vi "UMLEditor Main.vi"(1 "StartProject":string, 3 "StartTarget":string) -> ()   [LabVIEW 2020] (continued)
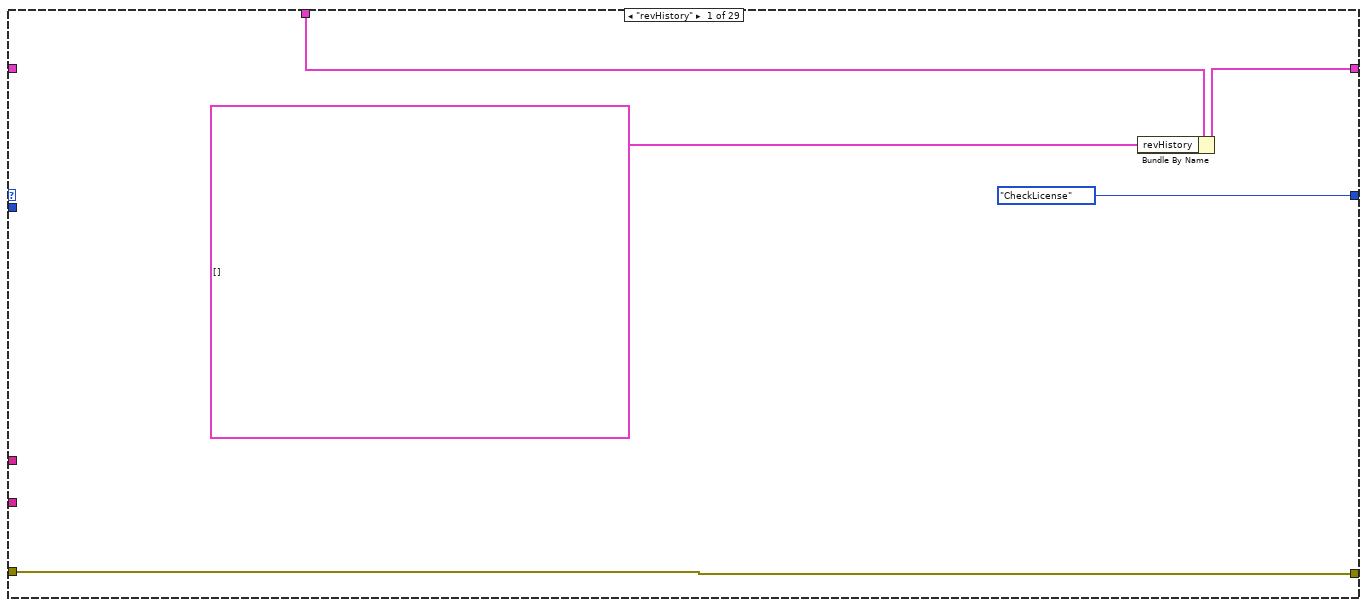
[diagram p8: hidden frame]
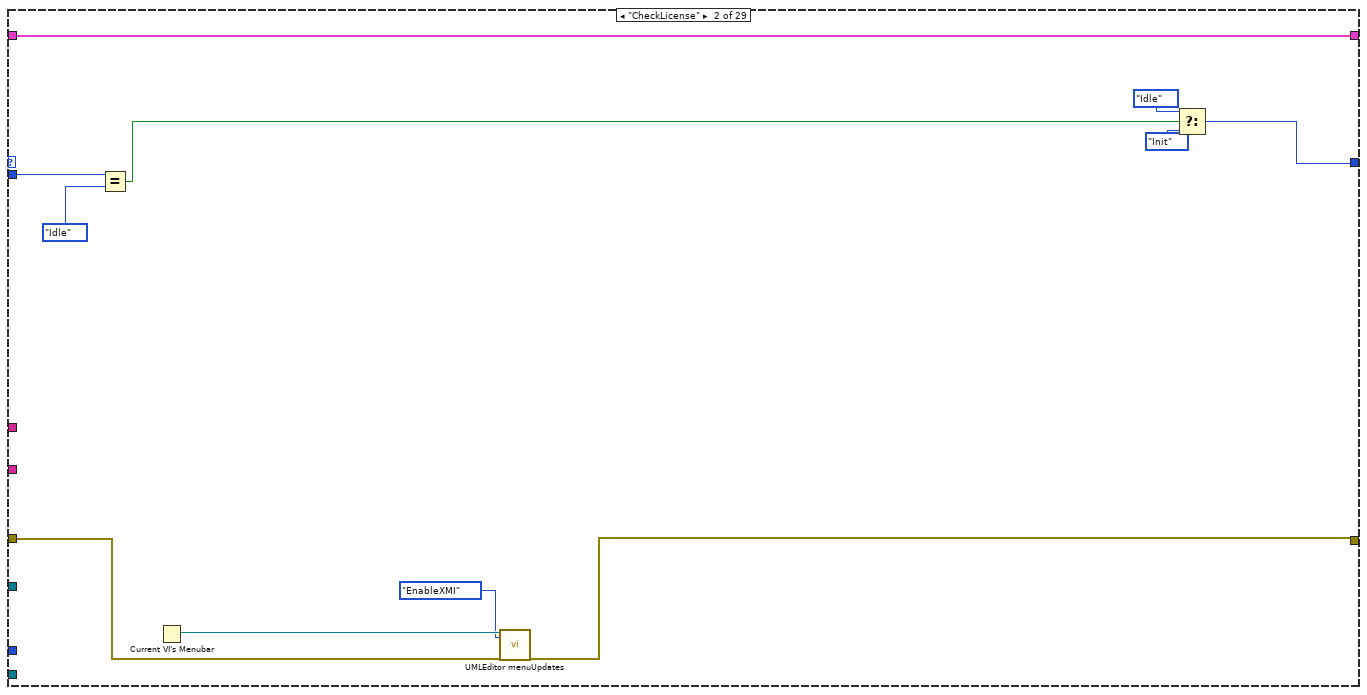
[diagram p9: hidden frame]
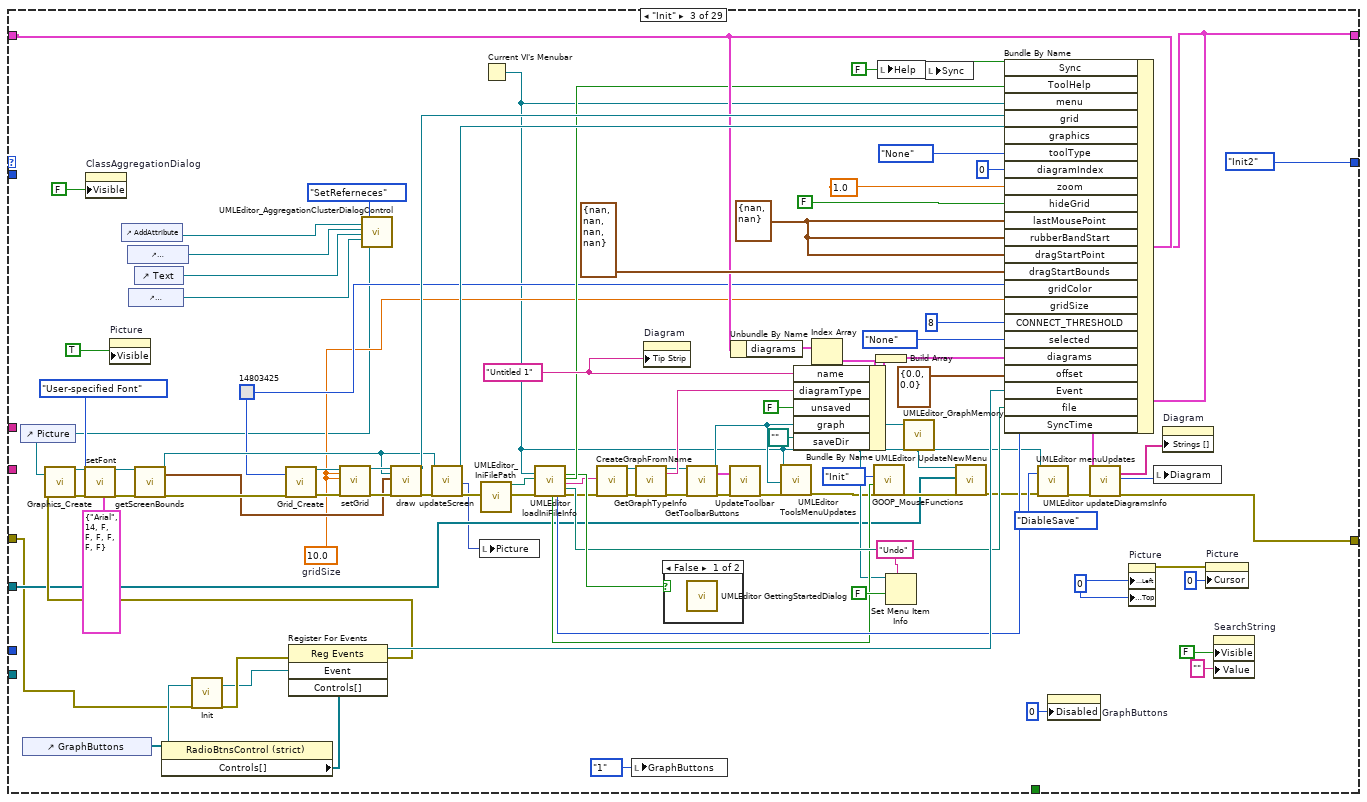
[diagram p10: hidden frame]
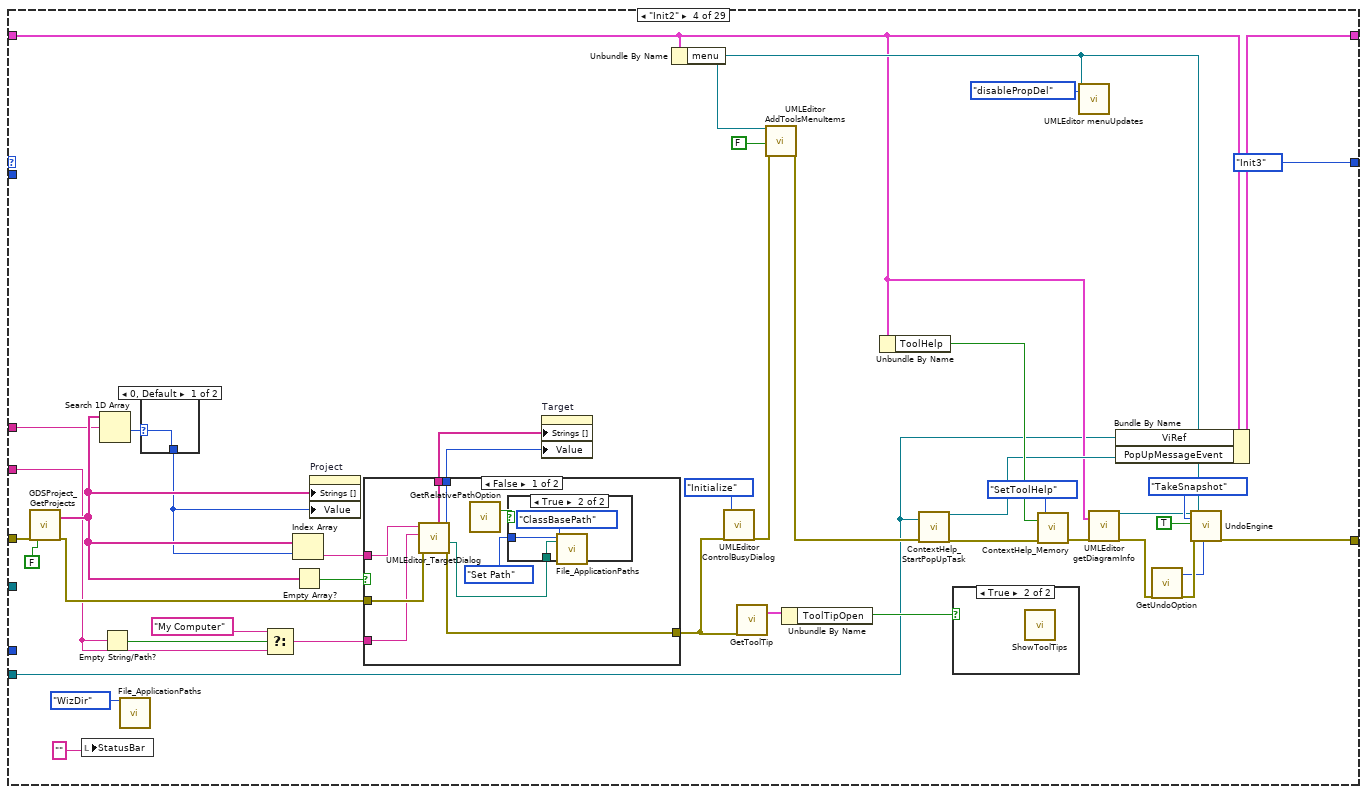
[diagram p12: hidden frame]
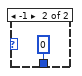
[diagram p14: hidden frame]
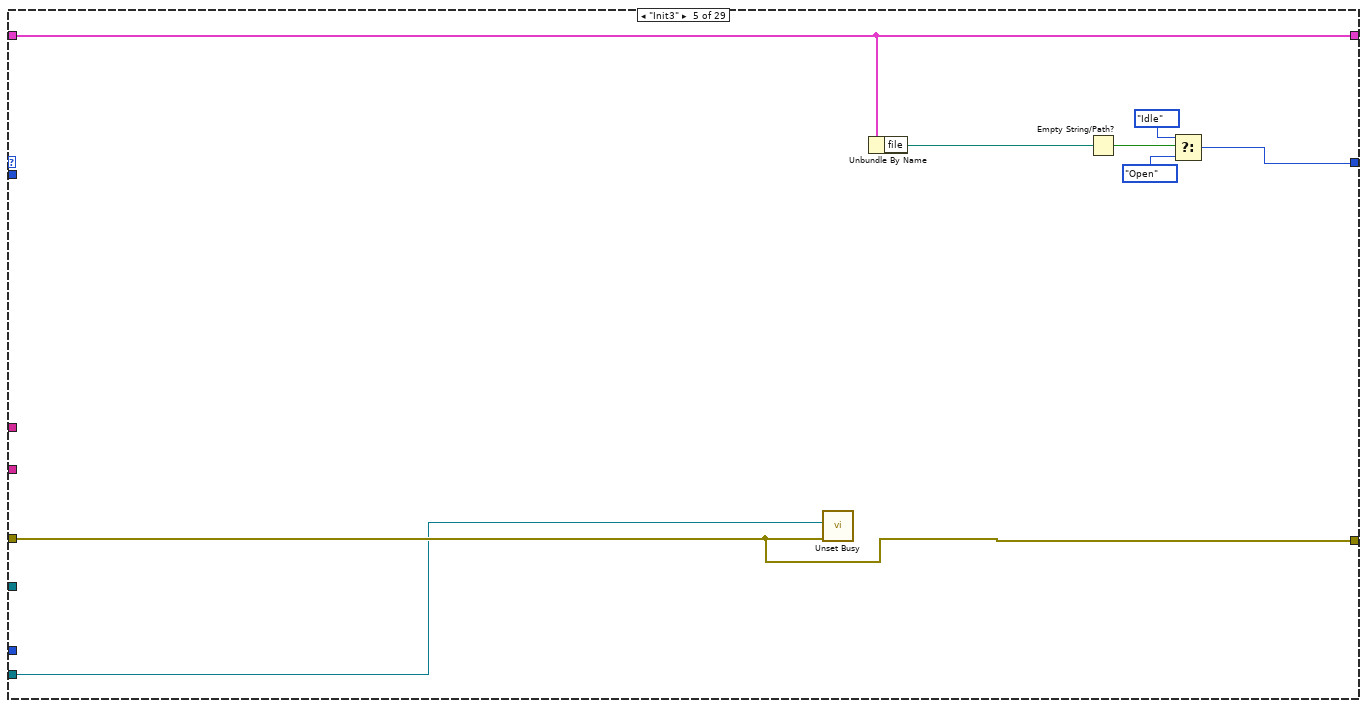
[diagram p17: hidden frame]
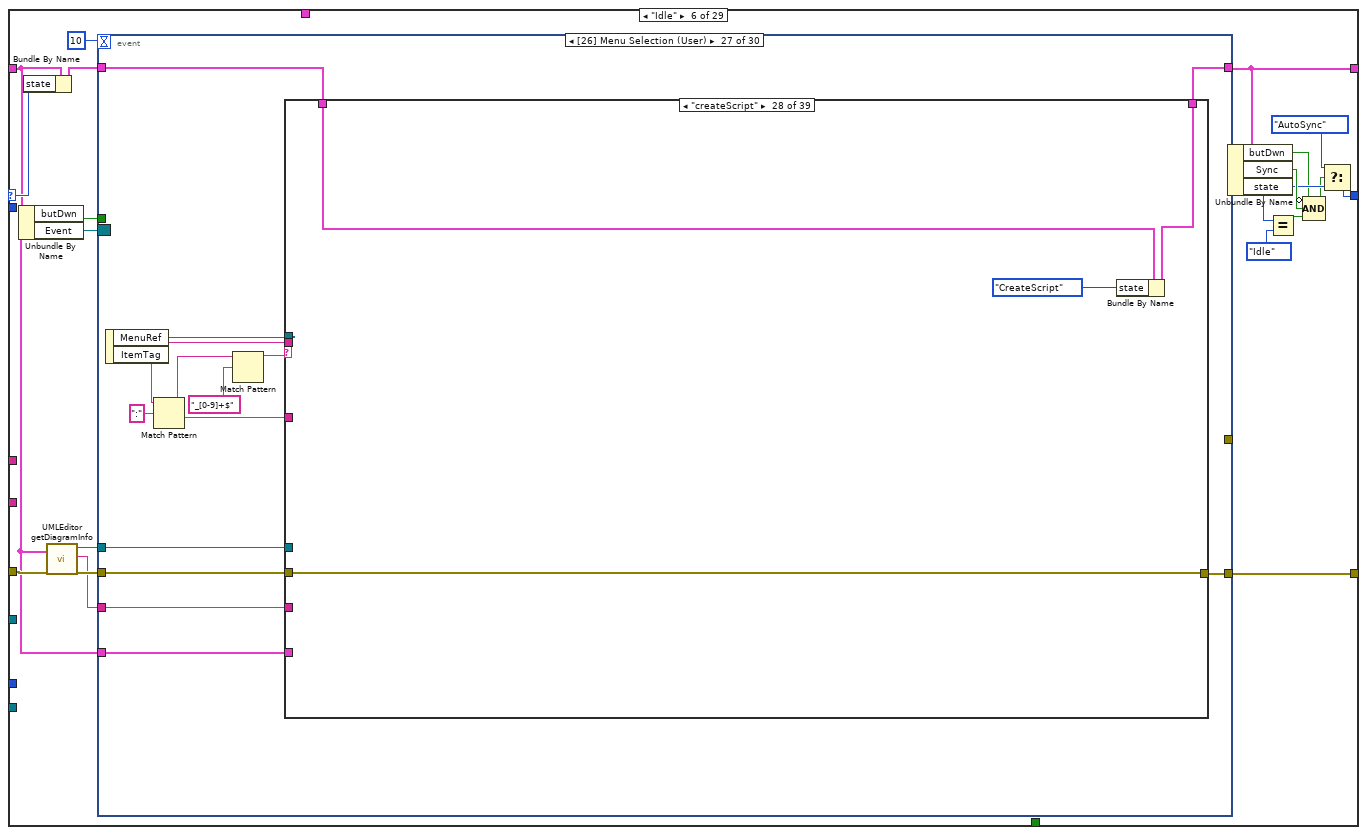
[diagram p18: hidden frame]
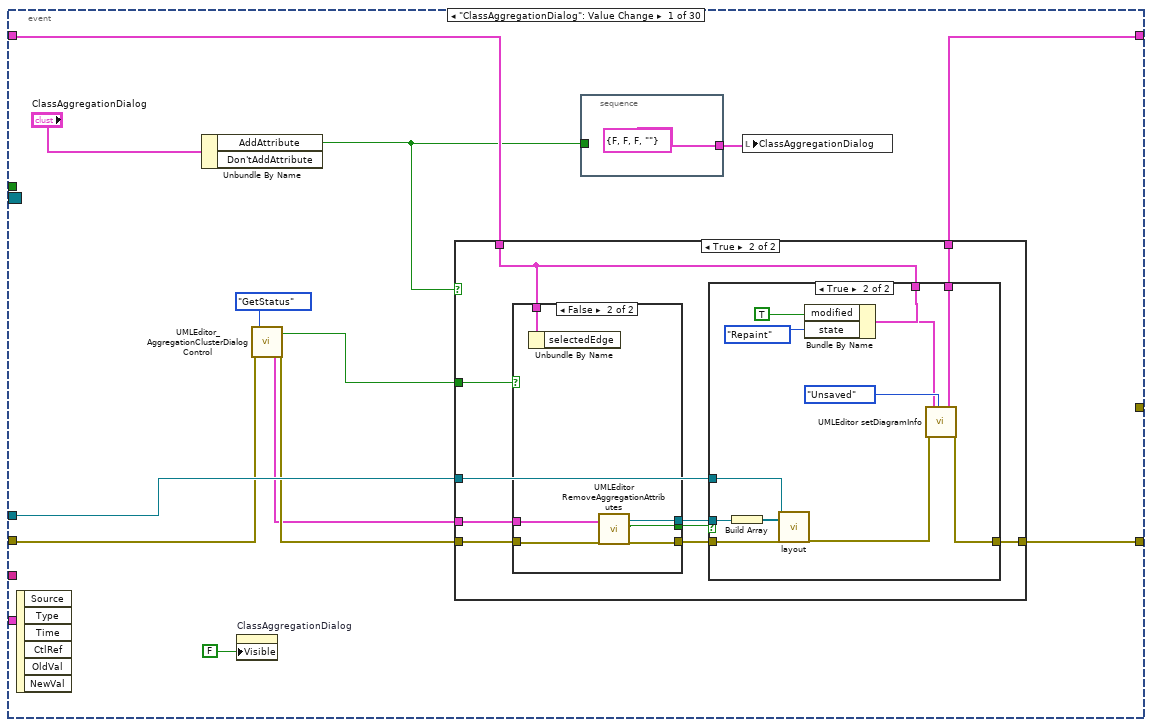
[diagram p19: hidden frame]
        n1897 = Unbundle By Name(w5102) -> ("lastMousePoint"=w5091:T9, "SelectedNodes"=w5098:refnum<class "AbstractNode.lvclass">[])
        n1898 = Unbundle By Name(w5102) -> ("graphics"=w5101:refnum<class "Graphics.lvclass">, "grid"=w5100:refnum<class "Grid.lvclass">)
        n1899 = call <resource>:"UMLEditor getDiagramInfo.vi"("localVariables"=w5102, "error in (no error)"=w5104) -> ("graph"=w5099:refnum<class "Graph.lvclass">, "error out"=w5097:errorcluster)  [unwired: 16 out]
        n1900 = call <resource>:"SelectPatternDialog.vi"("GraphIn"=w5099, "SelectedNodes"=w5098, "error in"=w5097) -> ("GraphOut"=w5092:refnum<class "Graph.lvclass">, "Cancelled"=w5095:bool, "NodesOut"=w5094:T57[], "LinksOut"=w5093:T59[], "NodeIndexies"=w5090:i32[], "error out"=w5096:errorcluster)  [unwired: 11 in]
        n1901 = case shown="False" w5095 {
          tunnel: w5096 -> [w5125 w5134]
          tunnel: [w5129 w5134] -> w5105
          tunnel: w5102 -> [w5110 w5133]
          tunnel: [w5131 w5133] -> w5103
          tunnel: w5101 -> [w5126 _]
          tunnel: w5100 -> [w5127 _]
          tunnel: w5094 -> [w5122 _]
          tunnel: w5093 -> [w5121 _]
          tunnel: w5092 -> [w5128 _]
          tunnel: w5091 -> [w5120 _]
          tunnel: w5090 -> [w5111 _]
          frame False {
            n1902 = Unbundle(w5120) -> ("x"=w5118:dbl, "y"=w5113:dbl)
            n1903 = Not A Number/Path/Refnum?(number/path/refnum=w5113) -> (NaN/Path/Refnum?=w5114:bool)
            n1904 = Not A Number/Path/Refnum?(number/path/refnum=w5118) -> (NaN/Path/Refnum?=w5119:bool)
            n1905 = Select(t=0.0, s=w5114, f=w5113) -> (s? t:f=w5112:dbl)
            n1906 = Select(t=0.0, s=w5119, f=w5118) -> (s? t:f=w5116:dbl)
            n1907 = call <resource>:"DesignPatterns_DrawNodesAndLinks.vi"("GraphIn"=w5128, "Graphics"=w5126, "Grid"=w5127, "Nodes"=w5122, "Links"=w5121, "error in (no error)"=w5125, "Y-Offset"=w5112, "NodeIndexies"=w5111, "X-Offset"=w5116) -> ("GraphOut"=w5123:refnum<class "Graph.lvclass">, "NodesCreated/Modified"=w5108:refnum<class "AbstractNode.lvclass">[], "error out"=w5124:errorcluster)  [unwired: 8 in]
            n1908 = Bundle By Name(cluster=w5110, "selected"=UMLEditor_tooltype."Node" ("selcted"), "SelectedNodes"=w5108) -> (w5109:T5)
            n1909 = call <resource>:"UMLEditor setDiagramInfo.vi"("error in (no error)"=w5124, "localVariablesIn"=w5109, "action"=enum16{"Name/Dir", "Unsaved", "Saved"}."Unsaved") -> ("localVariablesOut"=w5131:T5, "error out"=w5130:errorcluster)  [unwired: 2 in, 13 out]
            n1910 = call-dynamic "layout.vi"("reference"=w5123, "error in (no error)"=w5130) -> ("error out"=w5129:errorcluster)  [unwired: 16 in, 1 out]
          }
          frame True {
          }
        }
      }
      frame "SyncAll" {
        n1911 = Unbundle By Name(w5137) -> ("graphics"=w5146:refnum<class "Graphics.lvclass">, "grid"=w5145:refnum<class "Grid.lvclass">)
        n1912 = call <resource>:"UMLEditor getDiagramInfo.vi"("localVariables"=w5137, "error in (no error)"=w5160) -> ("graph"=w5159:refnum<class "Graph.lvclass">, "error out"=w5149:errorcluster)  [unwired: 16 out]
        n1913 = call-dynamic "getNodes.vi"("reference"=w5159, "error in (no error)"=w5149) -> ("reference out"=w5147:refnum<class "Graph.lvclass">, "nodes"=w5154:refnum<class "AbstractNode.lvclass">[], "error out"=w5155:errorcluster)  [unwired: 15 in]
        n1914 = Index Array(array=w5154) -> (element=w5158:refnum<class "AbstractNode.lvclass">)  [unwired: 1 in]
        n1915 = Initialize Array(w5158, 0 ("dimension size")) -> (w5156:refnum<class "AbstractNode.lvclass">[])
        n1916 = for {
          shift-right: [w5220] -> w5144
          shift-left: w5155 -> [w5222]
          tunnel: w5154 -> [w5221] mode=indexing
          shift-right: [w5217] -> w5150
          shift-left: w5156 -> [w5219]
          n1917 = call <resource>:"AbstractNode_GetObjectStatus.vi"("reference in"=w5221, "error in (no error)"=w5222) -> ("Class name"=w5216:string, "reference out"=w5218:refnum<class "AbstractNode.lvclass">, "error out"=w5220:errorcluster)  [unwired: 15 out]
          n1918 = case shown="\"ClassNode\", \"InterfaceNode\"" w5216 {
            tunnel: w5219 -> [w5223 w5226]
            tunnel: w5218 -> [_ w5225]
            tunnel: [w5223 w5224] -> w5217
            frame Default {
            }
            frame "ClassNode", "InterfaceNode" {
              n1919 = Build Array (concatenate)(w5226, w5225) -> (w5224:refnum<class "AbstractNode.lvclass">[])
            }
          }
        }
        n1920 = local read "StatusBar"() -> (w5138:string)
        n1921 = Equal?(x=w5142, y=UMLEditor_statesType."AutoSync") -> (x = y?=w5140:bool)
        n1922 = case shown="True" w5140 {
          tunnel: [_ w5169] -> w5135
          frame False {
          }
          frame True {
            n1923 = property on="Picture" class="Pict"("DisabledEnum"=T35."Disabled and Grayed Out" ("Disabled")) -> (error out=w5171:errorcluster)  [unwired: 2 in, 1 out]
            n1924 = call <vilib>:"Set Busy.vi"("error in (no error)"=w5171) -> ("error out"=w5169:errorcluster)  [unwired: 9 in, 1 out]
          }
        }
        n1925 = for {
          N -> [w5172]
          shift-right: [w5201] -> w5139
          shift-left: w5144 -> [w5195]
          tunnel: w5150 -> [w5182] mode=indexing
          tunnel: w5147 -> [w5198]
          tunnel: w5146 -> [w5197]
          tunnel: w5145 -> [w5196]
          shift-right: [w5184] -> _
          shift-left: path[] [] -> [w5184]
          tunnel: w5140 -> [w5179]
          tunnel: w5138 -> [_]
          i -> [w5176]
          stop <- w5180 stop-if-true
          n1926 = To More Specific Class(target class=refnum<class "ClassNode.lvclass"> refnum ("reference"), reference=w5182) -> (specific class reference=w5181:refnum<class "ClassNode.lvclass">)  [unwired: 1 in, 1 out]
          n1927 = call-dynamic "getClassInfo.vi"("reference"=w5181, "error in (no error)"=w5195) -> ("reference out"=w5194:refnum<class "ClassNode.lvclass">, "className"=w5191:string, "ClassPath"=w5192:path, "error out"=w5193:errorcluster)  [unwired: 8 in, 6 out]
          n1928 = Select(t=-1, s=w5179, f=w5176) -> (s? t:f=w5178:i32)
          n1929 = Empty String/Path?(string/path=w5192) -> (empty?=w5200:bool)
          n1930 = Not A Number/Path/Refnum?(number/path/refnum=w5192) -> (NaN/Path/Refnum?=w5199:bool)
          n1931 = Or(x=w5200, y=w5199) -> ()  [unwired: 1 out]
          n1932 = Increment(x=w5176) -> (x+1=w5173:i32)
          n1933 = call <resource>:"ReversedEngineering SyncUmlFromCode.vi"("SyncAction"=ReversedEngineering_SyncUmlFromCodeActions."GetAll", "ClassPath"=w5192, "NodeRef"=w5194, "GraphRef"=w5198, "IgnoreClasses"=w5184, "error in (no error)"=w5193, "ClassName(needed for lllbs)"=w5191, "graphics"=w5197, "IterationNo"=w5178, "grid"=w5196, "IterationsN"=w5172) -> ("Cancelled"=w5180:bool, "ClassName"=w5186:string, "attributes"=w5188:string, "methods"=w5187:string, "error out"=w5189:errorcluster)  [unwired: 1 in, 3 out]
          n1934 = Empty String/Path?(string/path=w5186) -> (empty?=w5185:bool)
          n1935 = case shown="False" w5185 {
            tunnel: w5189 -> [w5210 w5215]
            tunnel: w5188 -> [w5209 _]
            tunnel: w5187 -> [w5208 _]
            tunnel: [w5204 w5215] -> w5201
            tunnel: w5194 -> [w5203 _]
            tunnel: w5186 -> [w5202 _]
            frame False {
              n1936 = call-dynamic "ExternalSetParam.vi"("reference"=w5203, "setParameter"=ExternalSetTypes."Attributes", "string"=w5209, "error in (no error)"=w5210) -> ("reference out"=w5212:refnum<class "ClassNode.lvclass">, "error out"=w5213:errorcluster)  [unwired: 14 in]
              n1937 = call-dynamic "ExternalSetParam.vi"("reference"=w5212, "setParameter"=ExternalSetTypes."Methods", "string"=w5208, "error in (no error)"=w5213) -> ("reference out"=w5205:refnum<class "ClassNode.lvclass">, "error out"=w5206:errorcluster)  [unwired: 14 in]
              n1938 = call-dynamic "ExternalSetParam.vi"("reference"=w5205, "setParameter"=ExternalSetTypes."Name", "string"=w5202, "error in (no error)"=w5206) -> ("error out"=w5204:errorcluster)  [unwired: 14 in, 1 out]
            }
            frame True {
            }
          }
          n1939 = Format Into String(format string="Synchronizing %d of %d", w5173, w5172) -> (resulting string=w5174:string)  [unwired: 2 in, 1 out]
          n1940 = local write "StatusBar"(w5174) -> ()
        }
        n1941 = case shown="True" w5140 {
          tunnel: w5139 -> [_ _]
          tunnel: w5137 -> [w5163 w5166]
          tunnel: [w5163 w5165] -> w5136
          tunnel: w5135 -> [_ _]
          frame False {
          }
          frame True {
            n1942 = Get Date/Time In Seconds() -> (seconds since 1Jan1904=w5164:timestamp)
            n1943 = Bundle By Name(cluster=w5166, "LastSync"=w5164) -> (w5165:T5)
            n1944 = property on="Picture" class="Pict"("DisabledEnum"=T35."Enabled" ("Disabled")) -> (error out=w5167:errorcluster)  [unwired: 2 in, 1 out]
            n1945 = call <vilib>:"Unset Busy.vi"("error in (no error)"=w5167) -> ()  [unwired: 10 in, 1 out]
          }
        }
        n1946 = stacked-sequence {
          tunnel: w5139 -> [_]
          tunnel: w5138 -> [w5162]
          frame #0 {
            n1947 = local write "StatusBar"(w5162) -> ()
          }
        }
        n1948 = call <resource>:"UMLEditor setDiagramInfo.vi"("error in (no error)"=w5139, "localVariablesIn"=w5136, "action"=enum16{"Name/Dir", "Unsaved", "Saved"}."Unsaved") -> ("localVariablesOut"=w5151:T5, "error out"=w5153:errorcluster)  [unwired: 2 in, 13 out]
        n1949 = call-dynamic "layout.vi"("reference"=w5147, "error in (no error)"=w5153) -> ("error out"=w5148:errorcluster)  [unwired: 16 in, 1 out]
      }
      frame "StraightenAssociation" {
        n1950 = call <resource>:"UMLEditor getDiagramInfo.vi"("localVariables"=w5231, "error in (no error)"=w5239) -> ("graph"=w5238:refnum<class "Graph.lvclass">, "error out"=w5234:errorcluster)  [unwired: 16 out]
        n1951 = call-dynamic "getEdges.vi"("reference"=w5238, "error in (no error)"=w5234) -> ("reference out"=w5230:refnum<class "Graph.lvclass">, "edges"=w5233:refnum<class "AbstractEdge.lvclass">[], "error out"=w5232:errorcluster)  [unwired: 15 in]
        n1952 = Unbundle By Name(w5231) -> ("graphics"=w5229:refnum<class "Graphics.lvclass">, "grid"=w5228:refnum<class "Grid.lvclass">)
        n1953 = for {
          shift-right: [w5245] -> w5236
          shift-left: w5232 -> [w5248]
          tunnel: w5233 -> [w5247] mode=indexing
          tunnel: w5230 -> [w5243]
          tunnel: w5229 -> [w5242]
          tunnel: w5228 -> [w5241]
          n1954 = call-dynamic "StraightenAssociations.vi"("reference"=w5247, "error in (no error)"=w5248) -> ("reference out"=w5244:refnum<class "AbstractEdge.lvclass">, "error out"=w5246:errorcluster)  [unwired: 16 in]
          n1955 = call-dynamic "Layout.vi"("reference"=w5244, "graph"=w5243, "graphics"=w5242, "grid"=w5241, "error in (no error)"=w5246) -> ("error out"=w5245:errorcluster)  [unwired: 13 in, 1 out]
        }
        n1956 = call <resource>:"UMLEditor setDiagramInfo.vi"("error in (no error)"=w5236, "localVariablesIn"=w5231, "action"=enum16{"Name/Dir", "Unsaved", "Saved"}."Unsaved") -> ("localVariablesOut"=w5235:T5, "error out"=w5227:errorcluster)  [unwired: 2 in, 13 out]
      }
      frame "Exit" {
        # "Check if any unsaved"
        n1957 = Unbundle By Name(w5250) -> ("diagrams"=w5258:T8[])  [unwired: 1 out]
        n1958 = call <resource>:"UMLEditor getDiagramInfo.vi"("localVariables"=w5250) -> ("diagramType"=w5249:T27)  [unwired: 1 in, 17 out]
        n1959 = for {
          tunnel: w5258 -> [w5264] mode=indexing
          tunnel: [w5263] -> w5257 mode=indexing
          n1960 = Unbundle By Name(w5264) -> ("unsaved"=w5263:bool)
        }
        n1961 = Search 1D Array(1D array=w5257, element=TRUE) -> (index of element=w5254:i32)  [unwired: 1 out]
        n1962 = Bundle By Name(cluster=w5250, "quit"=TRUE ("element"), "diagramIndex"=w5254) -> (w5255:T5)
        n1963 = Greater Or Equal To 0?(x=w5254) -> (x >= 0?=w5253:bool)
        n1964 = Select(t=UMLEditor_statesType."Close" ("state"), s=w5253, f=UMLEditor_statesType."QUIT") -> (s? t:f=w5261:T6)
        n1965 = case shown="\"Idle\", Default" w5261 {
          tunnel: [w5265 w5268] -> w5262
          tunnel: w5251 -> [w5265 w5272]
          tunnel: w5255 -> [_ w5271]
          tunnel: w5249 -> [_ w5267]
          frame "Idle", Default {
          }
          frame "QUIT" {
            n1966 = call <resource>:"UMLEditor saveIniFileInfo.vi"("localVariables"=w5271, "error in (no error)"=w5272, "diagramType"=w5267) -> ("error out"=w5269:errorcluster)  [unwired: 16 out]
            n1967 = Unbundle By Name(w5269) -> ("code"=w5270:i32)
            n1968 = call <resource>:"UMLEditor_IniFilePath.vi"() -> ("Get Path"=w5266:path)  [unwired: 2 in, 17 out]
            n1969 = case shown="7, 8" w5270 {
              tunnel: w5269 -> [w5273 _]
              tunnel: [w5273 errorcluster {"status"=FALSE, "code"=0, "source"=""} ("error out")] -> w5268
              tunnel: w5266 -> [_ w5274]
              frame 0, Default {
              }
              frame 7, 8 {
                n1970 = Format Into String(format string="File permission error.\n\nMake sure the file to modify is writable.\n%s" ("message"), w5274) -> (resulting string=w5276:string)  [unwired: 2 in, 1 out]
                n1971 = One Button Dialog(message=w5276) -> ()  [unwired: 2 out]
              }
            }
          }
        }
      }
      frame "Error", Default {
        n1972 = Format Into String(w5281) -> (resulting string=w5280:string)  [unwired: 3 in, 1 out]
        n1973 = Unbundle By Name(w5278) -> ("code"=w5283:i32)
        n1974 = case shown="5011" w5283 {
          tunnel: [TRUE ("s") FALSE ("s") FALSE ("s") FALSE ("s") FALSE ("s") FALSE ("s") FALSE ("s") FALSE ("s") FALSE ("s") _ FALSE ("s")] -> w5282
          tunnel: w5280 -> [w5290 _ _ _ _ _ _ _ _ _ _]
          tunnel: w5279 -> [w5289 _ _ _ _ _ _ _ _ _ _]
          tunnel: w5278 -> [_ _ _ _ _ _ _ _ _ w5308 _]
          frame 0, Default {
            n1975 = call <resource>:"GDSError_LogErrorInformation.vi"("State"=w5290, "LocalVariableData"=w5289) -> ()  [unwired: 2 in, 16 out]
          }
          frame 1106, 1108 {
            n1976 = One Button Dialog(message="The saved file you tried to open,\nwas not compatible with this version.") -> ()  [unwired: 2 out]
          }
          frame 1044 {
            n1977 = One Button Dialog(message="A VI was locked, so the task has been stopped.") -> ()  [unwired: 2 out]
          }
          frame 1073 {
            n1978 = One Button Dialog(message="Trying to access a write protected file, or\na file that is currently running or reserved\nfor execution.") -> ()  [unwired: 2 out]
          }
          frame 56003 {
            n1979 = One Button Dialog(message="The new class(es) could not be added to the project since it would cause a conflict with an item already in memory.\n-This could be due to that the class created already exists in another opened project. Try to close other none used project to prevent this from happening.") -> ()  [unwired: 2 out]
          }
          frame 1025 {
            n1980 = One Button Dialog(message="The project reference is invalid.\nMake sure you have a selected project.") -> ()  [unwired: 2 out]
          }
          frame 1055 {
            n1981 = One Button Dialog(message="Class/Project reference error.\nThe reason for this could be:\n-The project has been closed\n-The class(es) has been removed from the project\n-The class(es) don't exist in the selected project") -> ()  [unwired: 2 out]
          }
          frame 7000 {
            n1982 = One Button Dialog(message="The class reference could not be obtained from the project.\nThe reason for this could be:\n-The project has been closed\n-The class has been removed from the project\n-The class don't exist in the selected project") -> ()  [unwired: 2 out]
          }
          frame 56001 {
            n1983 = One Button Dialog(message="Class(es) with the same name already exists in the project.") -> ()  [unwired: 2 out]
          }
          frame 5011 {
            n1984 = call <resource>:"GDSError_ReportError.vi"("error in (no error)"=w5308) -> ()  [unwired: 19 out]
          }
          frame 8 {
            n1985 = One Button Dialog(message="File permission error.\n\nMake sure the file to modify is writable.") -> ()  [unwired: 2 out]
          }
        }
        n1986 = Select(t=w5278, s=w5282, f=errorcluster {"status"=FALSE, "code"=0, "source"=""} ("error out")) -> (s? t:f=w5284:errorcluster)
        n1987 = Select(t=UMLEditor_statesType."QUIT" ("state"), s=w5282, f=UMLEditor_statesType."Idle" ("state")) -> (s? t:f=w5288:T6)
      }
    }
    n1988 = Select(t=UMLEditor_statesType."Error" ("state"), s=w60, f=w65) -> (s? t:f=w53:T6)
    n1989 = case shown="Error" w60 {
      frame No Error {
      }
      frame Error {
      }
    }
    n1990 = Equal?(x=w65, y=UMLEditor_statesType."QUIT" ("state")) -> (x = y?=w70:bool)
  }
  n1991 = Unbundle By Name(w31) -> ("graphics"=w40:refnum<class "Graphics.lvclass">, "grid"=w42:refnum<class "Grid.lvclass">, "diagrams"=w38:T8[])
  n1992 = for {
    shift-right: [w5312] -> w39
    shift-left: w28 -> [w5313]
    tunnel: w38 -> [w5314] mode=indexing
    n1993 = Unbundle By Name(w5314) -> ("graph"=w5311:refnum<class "Graph.lvclass">)
    n1994 = call-dynamic "Destroy.vi"("reference"=w5311, "error in (no error)"=w5313) -> ("error out"=w5312:errorcluster)  [unwired: 17 in]
  }
  n1995 = call-dynamic "Destroy.vi"("reference"=w42, "error in (no error)"=w39) -> ("error out"=w41:errorcluster)  [unwired: 16 in, 1 out]
  n1996 = call-dynamic "Destroy.vi"("reference"=w40, "error in (no error)"=w41) -> ("# of objects"=w33:i32)  [unwired: 16 in, 1 out]
  n1997 = case shown="Error" w28 {
    selector: w28 -> [w5315 w5316]
    tunnel: [w5315 w5316] -> w10
    tunnel: w31 -> [_ _]
    tunnel: w33 -> [_ _]
    frame No Error {
    }
    frame Error {
      n1998 = call <resource>:"GDSError_ReportError.vi"("error in (no error)"=w5316) -> ()  [unwired: 19 out]
    }
  }
  n1999 = Unbundle By Name(w31) -> ("Event"=w30:refnum<event-registration>)  [unwired: 1 out]
  n2000 = stacked-sequence {
    tunnel: w10 -> [w5326]
    tunnel: [w5326] -> w36
    tunnel: w30 -> [w5319]
    frame #0 {
      # "Kill Tasks"
      n2001 = call <resource>:"UMLEditor_SetMouseCursor.vi"("CursorType"=UMLEditor_Cursortype."Arrow") -> ("AllCursors"=w5318:refnum<k1>[])  [unwired: 9 in, 1 out]
      n2002 = call <resource>:"ContextHelp_StopPopUpTask.vi"() -> ()  [unwired: 2 in, 18 out]
      n2003 = call <resource>:"UMLEditor ClipBoard.vi"("menuAction"=UMLEditor_ClipBoardActionType."EmptyClipBoard") -> ()  [unwired: 5 in, 14 out]
      n2004 = call <resource>:"CleanUp.vi"() -> ()  [unwired: 1 in, 19 out]
      n2005 = call <resource>:"UMLEditor ControlBusyDialog.vi"("Action(SendStatusMessage)"=UMLEditor_BusyDialogAction."Quit" ("Action")) -> ()  [unwired: 3 in, 16 out]
      n2006 = for {
        tunnel: w5318 -> [w5327] mode=indexing
        n2007 = call <vilib>:"Destroy Cursor.vi"("cursor ID"=w5327) -> ()  [unwired: 1 in, 9 out]
      }
      n2008 = call <resource>:"CommonVIs_UmlOpenVIRef.vi"("ProjectNameIn"="clear" ("pattern (all files)")) -> ()  [unwired: 3 in, 8 out]
      n2009 = Unregister For Events(event registration refnum=w5319) -> ()  [unwired: 1 in, 1 out]
      n2010 = property on="SearchString" class="Str"("Visible"=FALSE, "Value"="" ("SearchString")) -> ()  [unwired: 2 in, 2 out]
      n2011 = call <resource>:"GOOP_MouseFunctions.vi"("Action(Read)"=enum16{"Init", "Read", "Close"}."Close") -> ()  [unwired: 8 in, 3 out]
    }
  }
  n2012 = call <resource>:"UMLEditor RemoveStaticObjects.vi"("error in (no error)"=w36) -> ("error out"=w23:errorcluster)  [unwired: 18 out]
  "error out" <- w23
  n2013 = property on="Time" class="DigNum (strict)"("Visible"=w25) -> ()  [unwired: 2 in, 2 out]
  n2014 = case shown="False" w24 {
    tunnel: w9 -> [w5331 _]
    tunnel: w23 -> [_ _]
    frame False {
      n2015 = invoke class="VI" method="FP.Close"(reference=w5331) -> (reference out=w5329:refnum<vi>, error out=w5330:errorcluster)  [unwired: 2 in, 1 out]
      n2016 = property on="Time" class="DigNum (strict)"("Visible"=FALSE) -> ()  [unwired: 2 in, 2 out]
      n2017 = Close Reference(reference=w5329, error in (no error)=w5330) -> ()  [unwired: 1 out]
    }
    frame True {
    }
  }
